vi "test-traj-generate-8-way.vi"() -> ()   [LabVIEW 2019]
uses:
  <vilib>/Rock Robotics/WPI/ThirdParty/JAS_Junk/TrajLib/Trajectory_Library.lvlib
  <vilib>/Rock Robotics/WPI/ThirdParty/JAS_Junk/TrajLib/TypeDef/DISPLAY_WEIGHTED_WAYPOINT.ctl
  <vilib>/Rock Robotics/WPI/ThirdParty/JAS_Junk/TrajLib/TypeDef/TRANSLATION2D.ctl
  <vilib>/Rock Robotics/WPI/ThirdParty/JAS_Junk/TrajLib/TypeDef/ROTATION2D.ctl
  <vilib>/Rock Robotics/WPI/ThirdParty/JAS_Junk/TrajLib/TypeDef/POSE2D.ctl
  <vilib>/Rock Robotics/WPI/ThirdParty/JAS_Junk/TrajLib/TypeDef/TRAJ_CONFIG.ctl
  <vilib>/Analysis/Matrix/Datatypes/RealMatrix.ctl
  <vilib>/Analysis/Matrix/NI_Matrix.lvlib
  <vilib>/Rock Robotics/WPI/ThirdParty/JAS_Junk/TrajLib/TypeDef/POSEwCURVATURE.ctl
  <vilib>/Rock Robotics/WPI/ThirdParty/JAS_Junk/TrajLib/TypeDef/TRAJECTORY.ctl
  <vilib>/Rock Robotics/WPI/ThirdParty/JAS_Junk/TrajLib/TypeDef/TRAJ_STATE.ctl
  <vilib>/Rock Robotics/WPI/ThirdParty/JAS_Junk/TrajLib/TypeDef/SPLINE.ctl
  <vilib>/Rock Robotics/WPI/ThirdParty/JAS_Junk/TrajLib/TypeDef/DISPLAY_WAYPOINT.ctl
panel:
  in  "Tab Control":T1(tab)
  in  "Interior WAYPOINTS":T2[](array[typedef])=[{"X"=1.5, "Y"=1.5}, {"X"=0.0, "Y"=0.0}, {"X"=-1.5, "Y"=-1.5}, {"X"=-3.0, "Y"=0.0}, {"X"=-1.5, "Y"=1.5}, {"X"=0.0, "Y"=0.0}, {"X"=1.5, "Y"=-1.5}] {"Y" format="%14.3f"; "X" format="%14.3f"}
  in  "Initial_Position":T3={"X"=3.0, "Y"=0.0, "ANGLE"=1.571} {"ANGLE" format="%13.3f"; "Y" format="%13.3f"; "X" format="%13.3f"}
  in  "Ending_Position":T3={"X"=3.0, "Y"=0.0, "ANGLE"=1.571} {"ANGLE" format="%13.3f"; "Y" format="%13.3f"; "X" format="%13.3f"}
  out "splines":T4[](array[typedef])
  out "ArrayPoseWithCurvature":T6[](array[typedef]) {"POSE"."ROTATION"."SIN" format="%13.4f"; "POSE"."ROTATION"."COS" format="%13.4f"; "POSE"."ROTATION"."VALUE" format="%13.4f"; "POSE"."TRANSLATION"."Y" format="%14.3f"; "POSE"."TRANSLATION"."X" format="%14.3f"}
  out "PoseCSize":i32
  out "error out 2":errorcluster
  in  "MaxVelocity":dbl=2.0 format="%17.4f"
  in  "MaxAcceleration":dbl=1.3 format="%17.4f"
  in  "TrackWidth_Meters":dbl=0.66 format="%20.4f"
  in  "Max Cent Accel":dbl=1.0 format="%20.4f"
  out "outTRAJECTORY_CONFIG":T9 {"End Velocity" format="%20.4f"; "StartVelocity" format="%20.4f"; "Max Acceleration" format="%20.4f"; "MaxVelocity" format="%20.4f"}
  out "TRAJECTORY":T10 {"States"."POSE"."ROTATION"."SIN" format="%13.4f"; "States"."POSE"."ROTATION"."COS" format="%13.4f"; "States"."POSE"."ROTATION"."VALUE" format="%13.4f"; "States"."POSE"."TRANSLATION"."Y" format="%14.3f"; "States"."POSE"."TRANSLATION"."X" format="%14.3f"; "TotalTImeSecs" format="%20.3f"}
  out "size(s)":i32
  out "error out":errorcluster
  out "read Traj":errorcluster
  out "readTRAJECTORY":T10 {"States"."POSE"."ROTATION"."SIN" format="%13.4f"; "States"."POSE"."ROTATION"."COS" format="%13.4f"; "States"."POSE"."ROTATION"."VALUE" format="%13.4f"; "States"."POSE"."TRANSLATION"."Y" format="%14.3f"; "States"."POSE"."TRANSLATION"."X" format="%14.3f"; "TotalTImeSecs" format="%20.3f"}
  out "size(s) 2":i32
  out "file write error":errorcluster
  out "appended path":path
  out "XY Graph":cluster{dbl[], dbl[]}(graph)
  out "Position":cluster{dbl[], dbl[]}(graph)
  out "Time":dbl
  in  "STEP":bool
  out "XY Graph 2":cluster{dbl[], dbl[]}(graph)
  out "TimeSeconds":dbl
  out "OutputTRAJ_STATE":T11={"TimeSeconds"=0.0, "Velocity"=0.0, "Acceleration"=0.0, "POSE"={"TRANSLATION"={"X"=0.0, "Y"=0.0}, "ROTATION"={"VALUE"=0.0, "COS"=1.0, "SIN"=0.0}}, "Curvature"=0.0} {"POSE"."ROTATION"."SIN" format="%13.4f"; "POSE"."ROTATION"."COS" format="%13.4f"; "POSE"."ROTATION"."VALUE" format="%13.4f"; "POSE"."TRANSLATION"."Y" format="%14.3f"; "POSE"."TRANSLATION"."X" format="%14.3f"}
  in  "CONT":bool
  out "Done":bool
  # "Single step\nthrough \ntrajectory"
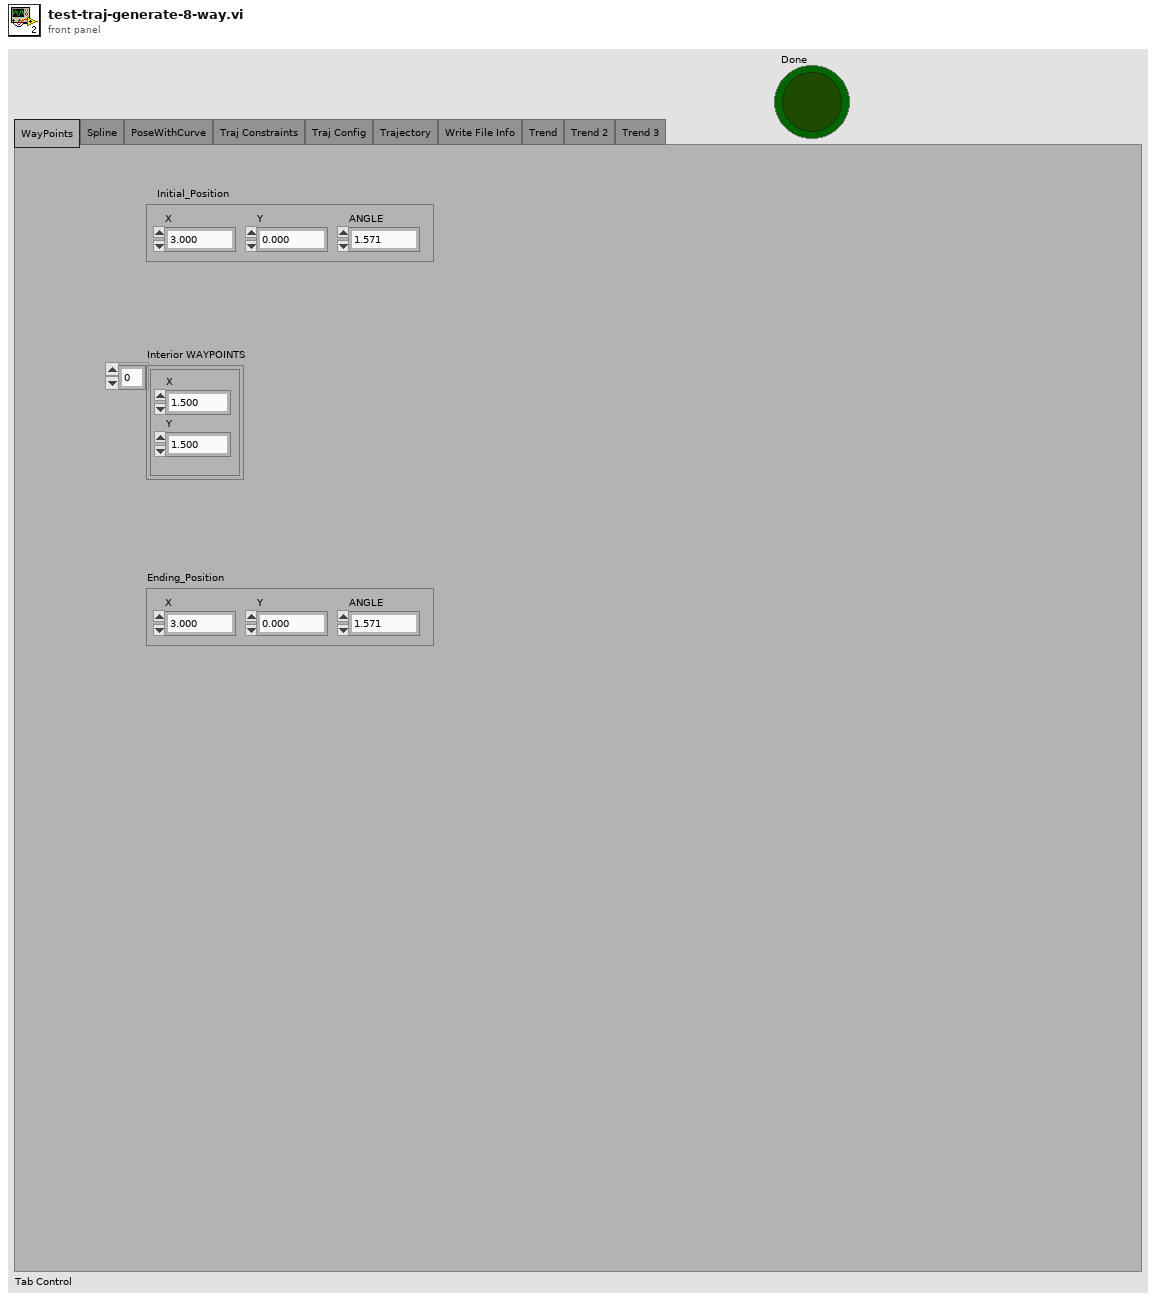
[diagram p1: front panel]
types:
  T1 = enum32{"WayPoints", "Spline", "PoseWithCurve", "Traj Constraints", "Traj Config", "Trajectory", "Write File Info", "Trend", "Trend 2", "Trend 3"}
  T2 = typedef "Trajectory_Library.lvlib/TRANSLATION2D.ctl" = cluster{"X":dbl, "Y":dbl}
  T3 = typedef "Trajectory_Library.lvlib/DISPLAY_WAYPOINT.ctl" = cluster{"X":dbl, "Y":dbl, "ANGLE":dbl}
  T4 = typedef "Trajectory_Library.lvlib/SPLINE.ctl" = cluster{"Degree":i32, "Coefficients":T5}
  T5 = typedef "NI_Matrix.lvlib/RealMatrix.ctl" = dbl[][]
  T6 = typedef "Trajectory_Library.lvlib/POSEwCURVATURE.ctl" = cluster{"CURVATURE":dbl, "POSE":T7}
  T7 = typedef "Trajectory_Library.lvlib/POSE2D.ctl" = cluster{"TRANSLATION":T2, "ROTATION":T8}
  T8 = typedef "Trajectory_Library.lvlib/ROTATION2D.ctl" = cluster{"VALUE":dbl, "COS":dbl, "SIN":dbl}
  T9 = typedef "Trajectory_Library.lvlib/TRAJ_CONFIG.ctl" = cluster{"MaxVelocity":dbl, "Max Acceleration":dbl, "StartVelocity":dbl, "End Velocity":dbl, "Reversed":bool, "Constraints":variant[]}
  T10 = typedef "Trajectory_Library.lvlib/TRAJECTORY.ctl" = cluster{"TotalTImeSecs":dbl, "States":T11[]}
  T11 = typedef "Trajectory_Library.lvlib/TRAJ_STATE.ctl" = cluster{"TimeSeconds":dbl, "Velocity":dbl, "Acceleration":dbl, "POSE":T7, "Curvature":dbl}
  T12 = typedef "Trajectory_Library.lvlib/DISPLAY_WEIGHTED_WAYPOINT.ctl" = cluster{"X":dbl, "Y":dbl, "ANGLE":dbl, "WEIGHT":dbl}
  T13 = typedef "Trajectory_Library.lvlib/DIFF_DRIVE_KINEMATICS.ctl" = cluster{"TrackWidth_Meters":dbl}
  T14 = typedef "Trajectory_Library.lvlib/SPLINE_CTRL_VECTOR.ctl" = cluster{"Xs":dbl[], "Ys":dbl[]}
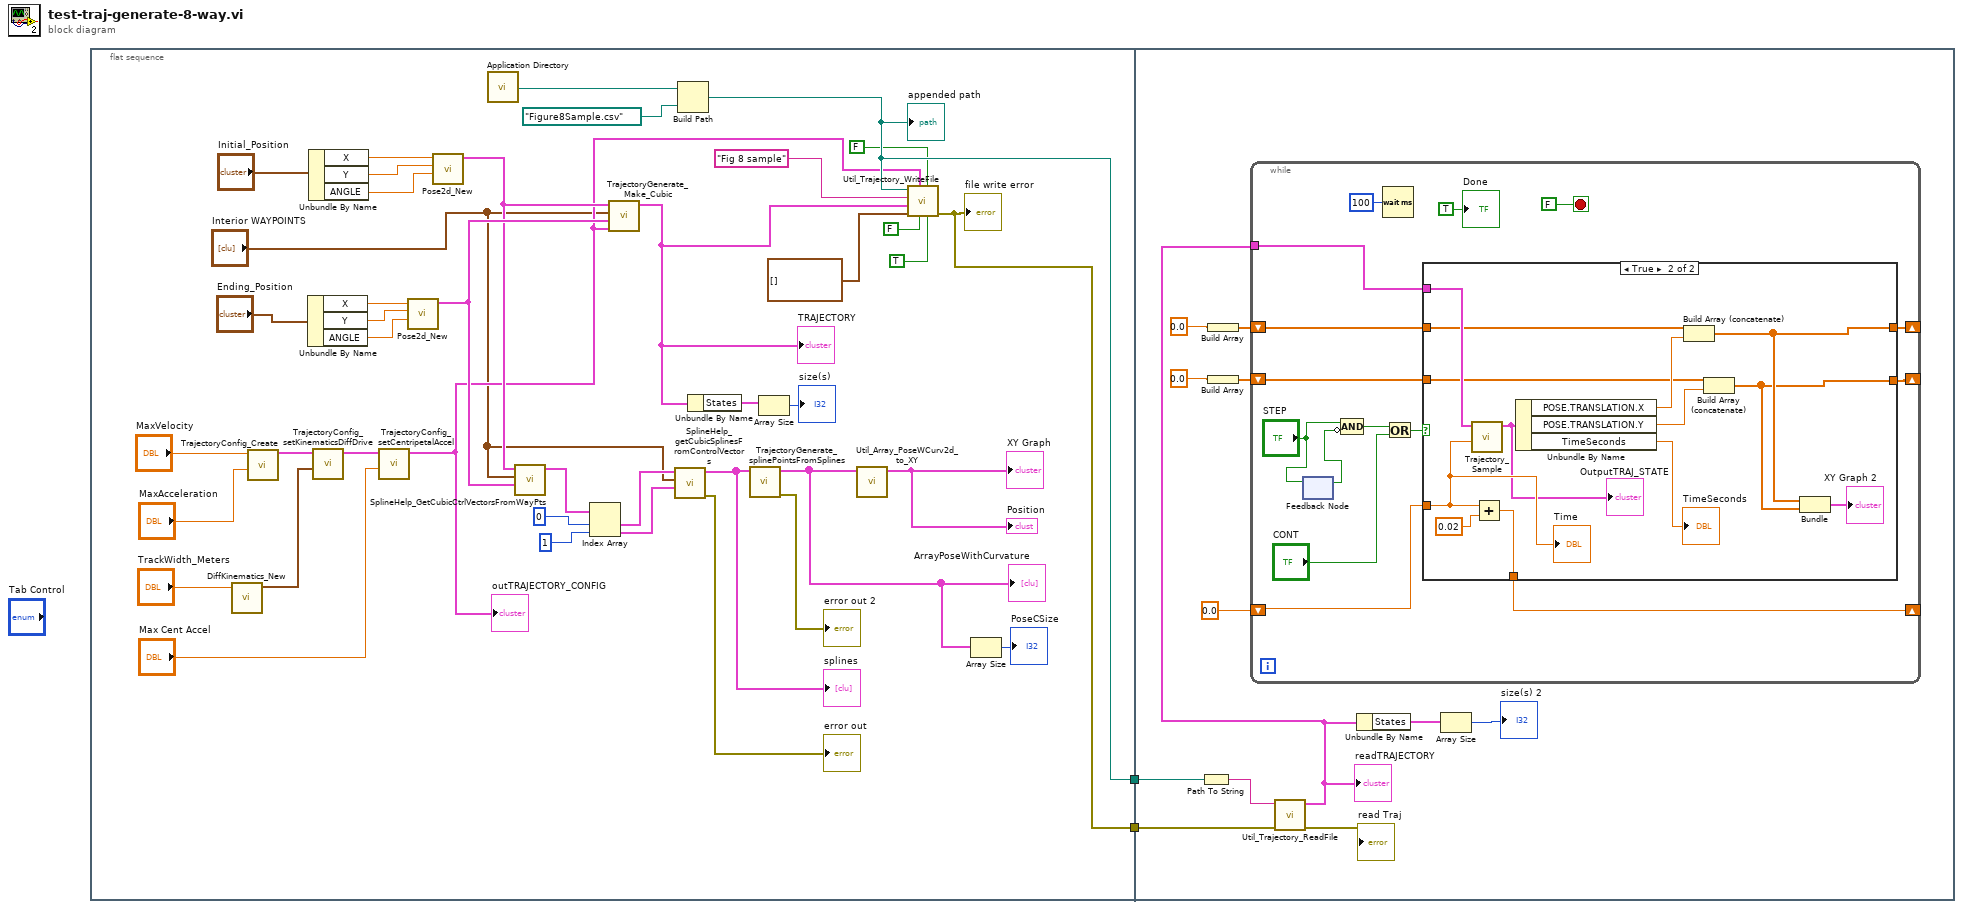
[diagram p0: block diagram]
diagram:
  n1 = flat-sequence {
    tunnel: [w11] -> w2
    tunnel: [w3] -> w1
    tunnel: w2 -> [w49]
    tunnel: w1 -> [w45]
    frame #0 {
      n2 = call <vilib>:"DiffKinematics_New.vi"("TrackWidth_Meters"="TrackWidth_Meters") -> ("DIFF_DRIVE_KINEMATICS"=w16:T13)  [unwired: 10 in]
      n3 = call <vilib>:"TrajectoryConfig_Create.vi"("MaxAcceleration"="MaxAcceleration", "MaxVelocity"="MaxVelocity") -> ("TRAJECTORY_CONFIG"=w18:T9)  [unwired: 9 in]
      n4 = Unbundle By Name("Ending_Position") -> ("X"=w40:dbl, "Y"=w39:dbl, "ANGLE"=w38:dbl)
      n5 = Unbundle By Name("Initial_Position") -> ("X"=w43:dbl, "Y"=w42:dbl, "ANGLE"=w41:dbl)
      n6 = call <vilib>:"TrajectoryConfig_setKinematicsDiffDrive.vi"("DIFF_DRIVE_KINEMATICS"=w16, "inTRAJECTORY_CONFIG"=w18) -> ("outTRAJECTORY_CONFIG"=w15:T9)  [unwired: 9 in]
      n7 = call <vilib>:"TrajectoryConfig_setCentripetalAccel.vi"("Max Cent Accel"="Max Cent Accel", "inTRAJECTORY_CONFIG"=w15) -> ("outTRAJECTORY_CONFIG"=w10:T9)  [unwired: 9 in]
      "outTRAJECTORY_CONFIG" <- w10
      n8 = call <vilib>:"Pose2d_New.vi"("Heading"=w38, "Y"=w39, "X"=w40) -> ("out POSe"=w36:T7)  [unwired: 8 in]
      n9 = call <vilib>:"Pose2d_New.vi"("Heading"=w41, "Y"=w42, "X"=w43) -> ("out POSe"=w35:T7)  [unwired: 8 in]
      n10 = call <vilib>:"Application Directory.vi"() -> ("Application Directory"=w12:path)
      n11 = call <vilib>:"SplineHelp_GetCubicCtrlVectorsFromWayPts.vi"("Enging POSE"=w36, "Interior WAYPOINTS"="Interior WAYPOINTS", "Starting POSE"=w35) -> ("SplineControlVectors"=w25:T14[])  [unwired: 8 in]
      n12 = Index Array(array=w25, index #1=0 ("index"), index #2=1 ("index")) -> (element #1=w24:T14, element #2=w23:T14)
      n13 = call <vilib>:"TrajectoryGenerate_Make_Cubic.vi"("traj_config"=w10, "Enging POSE"=w36, "Interior WAYPOINTS"="Interior WAYPOINTS", "Starting POSE"=w35) -> ("TRAJECTORY"=w22:T10)  [unwired: 6 in, 1 out]
      "TRAJECTORY" <- w22
      n14 = call <vilib>:"SplineHelp_getCubicSplinesFromControlVectors.vi"("endCtrlVector"=w23, "InternalWaypoints"="Interior WAYPOINTS", "startCtrlVector"=w24) -> ("error out"=→"error out":errorcluster, "splines"=w33:T4[])  [unwired: 3 in, 4 out]
      "splines" <- w33
      n15 = Build Path(base path=w12, name or relative path=path "Figure8Sample.csv" ("Trajectory File Name")) -> (appended path=w11:path)
      "appended path" <- w11
      n16 = Unbundle By Name(w22) -> ("States"=w31:T11[])
      n17 = call <vilib>:"TrajectoryGenerate_splinePointsFromSplines.vi"("inputSPLINE"=w33) -> ("error out"=→"error out 2":errorcluster, "ArrayPoseWithCurvature"=w8:T6[])  [unwired: 9 in]
      "ArrayPoseWithCurvature" <- w8
      n18 = Array Size(array=w31) -> (size(s)=→"size(s)":i32)
      n19 = call <vilib>:"Util_Array_PoseWCurv2d_to_XY.vi"("inArrayPoseWCurve"=w8) -> ("outArrayXY"=→"XY Graph" →"Position":cluster{dbl[], dbl[]})  [unwired: 10 in]
      n20 = call <vilib>:"Util_Trajectory_WriteFile.vi"("Trajectory is Cubic"=TRUE, "UseWeights"=FALSE, "Trajectory Is Relative"=FALSE, "TRAJECTORY_CONFIG"=w10, "UtilityWayPoints"=T12[] [], "TRAJECTORY"=w22, "Comment"="Fig 8 sample", "Trajectory File Name"=w11) -> ("error out"=w3:errorcluster)  [unwired: 3 in]
      "file write error" <- w3
      n21 = Array Size(array=w8) -> (size(s)=→"PoseCSize":i32)
    }
    frame #1 {
      n22 = Path To String(path=w49) -> (string=w50:string)
      n23 = Build Array(0.0) -> (w53:dbl[])
      n24 = Build Array(0.0) -> (w52:dbl[])
      n25 = call <vilib>:"Util_Trajectory_ReadFile.vi"("error in (no error)"=w45, "FileName"=w50) -> ("error out"=→"read Traj":errorcluster, "outTRAJECTORY"=w46:T10)  [unwired: 7 in, 1 out]
      "readTRAJECTORY" <- w46
      n26 = while {
        shift-right: [w67] -> _
        shift-left: 0.0 -> [w68]
        tunnel: w46 -> [w64]
        shift-right: [w63] -> _
        shift-left: w53 -> [w66]
        shift-right: [w62] -> _
        shift-left: w52 -> [w65]
        stop <- FALSE stop-if-true
        n27 = feedback-in #1("STEP") -> ()
        n28 = feedback #1() -> (w60:bool)  [unwired: 1 in]
        n29 = Compound Arithmetic op=AND("STEP", invert w60) -> (w58:bool)
        n30 = Wait (ms)(milliseconds to wait=u32 100) -> ()  [unwired: 1 out]
        n31 = Or(x=w58, y="CONT") -> (x .or. y?=w59:bool)
        n32 = case shown="True" w59 {
          tunnel: w68 -> [w74 w85]
          tunnel: [w74 w87] -> w67
          tunnel: w66 -> [w73 w81]
          tunnel: w65 -> [w72 w79]
          tunnel: w64 -> [_ w84]
          tunnel: [w73 w76] -> w63
          tunnel: [w72 w75] -> w62
          frame False {
          }
          frame True {
            n33 = call <vilib>:"Trajectory_Sample.vi"("Time"=w85, "InputTRAJECTORY"=w84) -> ("OutputTRAJ_STATE"=w83:T11)  [unwired: 9 in]
            "OutputTRAJ_STATE" <- w83
            n34 = Add(x=w85, y=0.02) -> (x+y=w87:dbl)
            n35 = Unbundle By Name(w83) -> ("POSE.TRANSLATION.X"=w80:dbl, "POSE.TRANSLATION.Y"=w78:dbl, "TimeSeconds"=→"TimeSeconds":dbl)
            n36 = Build Array (concatenate)(w81, w80) -> (w76:dbl[])
            n37 = Build Array (concatenate)(w79, w78) -> (w75:dbl[])
            n38 = Bundle(w76, w75) -> (→"XY Graph 2":cluster{dbl[], dbl[]})  [unwired: 1 in]
            "Time" <- w85
          }
        }
        "Done" <- TRUE ("Done")
      }
      n39 = Unbundle By Name(w46) -> ("States"=w48:T11[])
      n40 = Array Size(array=w48) -> (size(s)=→"size(s) 2":i32)
    }
  }
